vi "Measure Battery.vi"(0 "instrument handle":refnum<k15>, 11 "error in":errorcluster) -> (4 "instrument handle out":refnum<k15>, 6 "Measurement":T1, 15 "error out":errorcluster)   [LabVIEW 2026]
doc: "Full measurement of the cell on the given NI-DMM session (spec.txt, Measurement principle): (1) DC volts 10 V range 6.5 digits, input resistance above 10 GOhm, 10 readings give V1 and OCV Std Dev; (2) waveform 10 V 100 kS/s 20000 points gives Ripple pp (max - min) and Ripple RMS (std dev); (3) only when 0.2 V <= V1 <= 1.8 V: Diode function 10 V 6.5 digits (1 mA), mean of 5 readings gives Diode Voltage, then DC volts again gives V2, Internal Resistance = (Diode Voltage - (V1+V2)/2)/0.001 Ohm, +Inf when the diode reading is over-range or 4.0 V or more (the driver's over-range warning is not passed on as an error). Otherwise Diode Voltage and Internal Resistance are NaN. OCV is ALWAYS V1, the reading BEFORE the diode step, in both cases: V2 only cancels drift in the IR calculation, because the 1 mA diode current pumps up a regulated Li-ion cell and V2 then reads too high. The over-range warning (1073356801) is cleared from error out. Leaves the DMM in DC volts, single point. Does not open or close the session."
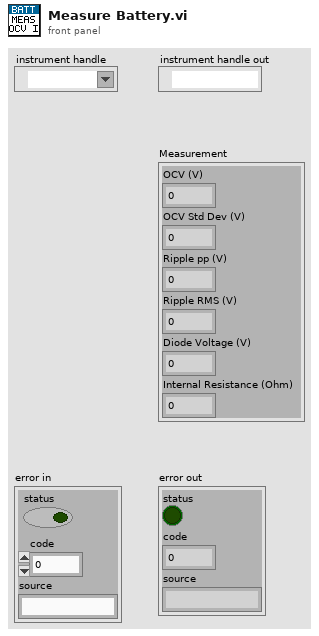
[diagram p1: front panel]
types:
  T1 = cluster{"OCV (V)":dbl, "OCV Std Dev (V)":dbl, "Ripple pp (V)":dbl, "Ripple RMS (V)":dbl, "Diode Voltage (V)":dbl, "Internal Resistance (Ohm)":dbl}
  T2 = enum16{"Immediate", "External", "TTL 0", "TTL 1", "TTL 2", "TTL 3", "TTL 4", "TTL 5", "TTL 6", "Interval", "Software", "TTL 7", "PXI Star", "LBR Trig 1", "Aux Trig 1"}
  T3 = enum16{"DC Volts", "AC Volts", "DC Current", "AC Current", "2-wire Resistance", "4-wire Resistance", "Diode", "Frequency", "Period", "AC Volts DC Coupled", "Capacitance", "Inductance", "Temperature"}
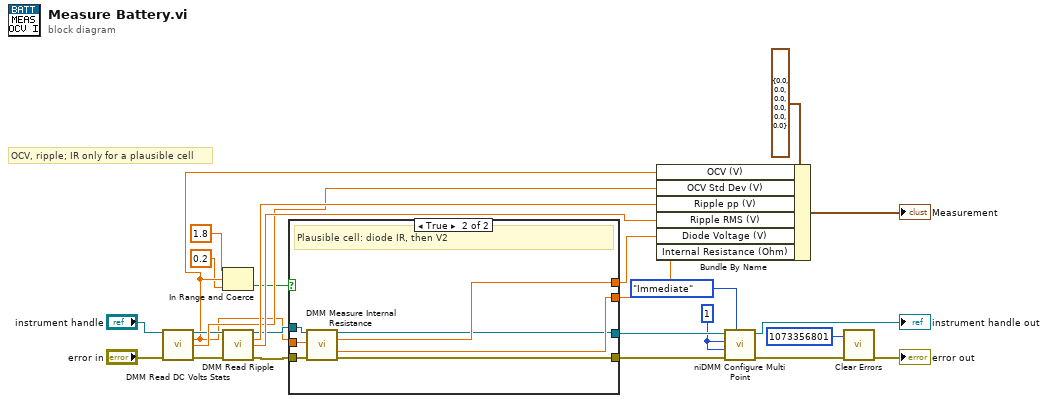
[diagram p0: block diagram]
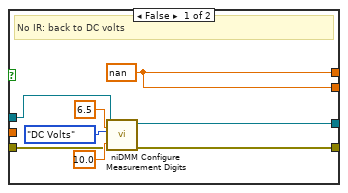
[diagram p2: hidden frame]
diagram:
  w8 = 1 ("Count")
  # "OCV, ripple; IR only for a plausible cell"
  n1 = call "DMM Read DC Volts Stats.vi"("instrument handle"="instrument handle", "error in"="error in") -> ("instrument handle out"=w20:refnum<k15>, "Mean (V)"=w13:dbl, "Std Dev (V)"=w21:dbl, "error out"=w22:errorcluster)  [unwired: 10 in]
  n2 = In Range and Coerce(upper limit=1.8, x=w13, lower limit=0.2) -> (In Range?=w12:bool)  [unwired: 1 out]
  n3 = call "DMM Read Ripple.vi"("instrument handle"=w20, "error in"=w22) -> ("instrument handle out"=w14:refnum<k15>, "Ripple pp (V)"=w23:dbl, "Ripple RMS (V)"=w24:dbl, "error out"=w15:errorcluster)  [unwired: 10 in]
  n4 = case shown="True" w12 {
    tunnel: [w30 w39] -> w18
    tunnel: [w30 w40] -> w19
    tunnel: w13 -> [_ w34]
    tunnel: w14 -> [w26 w35]
    tunnel: w15 -> [w27 w36]
    tunnel: [w28 w37] -> w16
    tunnel: [w29 w38] -> w17
    frame False {
      w30 = nan ("not measured")
      # "No IR: back to DC volts"
      n5 = call <instrlib>:"niDMM Configure Measurement Digits.vi"("Range"=10.0, "Resolution in Digits"=6.5, "error in (no error)"=w27, "Function"=T3."DC Volts", "instrument handle"=w26) -> ("error out"=w29:errorcluster, "instrument handle out"=w28:refnum<k15>)  [unwired: 5 in]
    }
    frame True {
      # "Plausible cell: diode IR, then V2"
      n6 = call "DMM Measure Internal Resistance.vi"("instrument handle"=w35, "V1 (V)"=w34, "error in"=w36) -> ("instrument handle out"=w37:refnum<k15>, "Diode Voltage (V)"=w39:dbl, "Internal Resistance (Ohm)"=w40:dbl, "error out"=w38:errorcluster)  [unwired: 8 in, 1 out]
    }
  }
  n7 = Bundle By Name(cluster=T1 {"OCV (V)"=0.0, "OCV Std Dev (V)"=0.0, "Ripple pp (V)"=0.0, "Ripple RMS (V)"=0.0, "Diode Voltage (V)"=0.0, "Internal Resistance (Ohm)"=0.0} ("Measurement"), "OCV (V)"=w13, "OCV Std Dev (V)"=w21, "Ripple pp (V)"=w23, "Ripple RMS (V)"=w24, "Diode Voltage (V)"=w18, "Internal Resistance (Ohm)"=w19) -> (→"Measurement":T1)
  n8 = call <instrlib>:"niDMM Configure Multi Point.vi"("Sample Trigger"=T2."Immediate", "error in (no error)"=w17, "Sample Count"=w8, "Trigger Count"=w8, "instrument handle"=w16) -> ("error out"=w25:errorcluster, "instrument handle out"=→"instrument handle out":refnum<k15>)  [unwired: 5 in]
  n9 = call <vilib>:"Clear Errors.vi"("error in (no error)"=w25, "specific error code to clear (0: all)"=1073356801 ("specific error code to clear")) -> ("error out"=→"error out":errorcluster)  [unwired: 4 in, 1 out]
